vi "Smart IO Set Led Device Buffer.vi"(6 "force":bool, 8 "error in (no error)":errorcluster, 9 "buffer Data":u32[](array[colorbox]), 11 "deviceIndex":i32=-1) -> (0 "error out":errorcluster)   [LabVIEW 2023, in "MrcLib.lvlib"]
doc: "Update the LED color buffer for the wired device channel or leave device unwired if you choose to update the entire buffer in a single call."
uses:
  <vilib>/MRC/MrcLib.lvlib
  <vilib>/MRC/Types/MRC Smart IO Mode.ctl
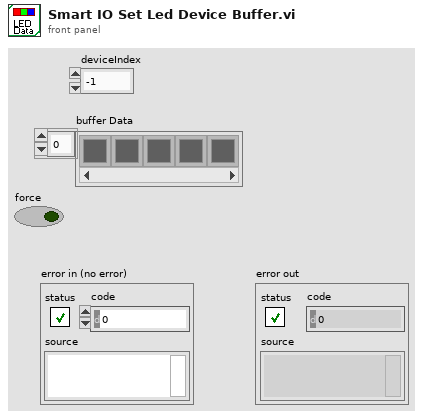
[diagram p1: front panel]
types:
  T1 = typedef "MRC Smart IO Mode.ctl" = i32
  T2 = enum16{"update device span", "update LED buffer", "clear"}
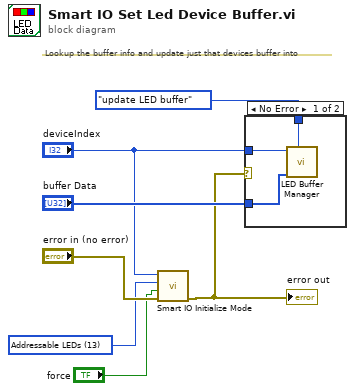
[diagram p0: block diagram]
diagram:
  w3 = T1 13 items=["Digital Input"=0, "Digital Output"=1, "Analog Input"=2, "PWM Input"=3, "PWM Output"=4, "Counter Rising"=5, "Counter Falling"=6, "Addressable LEDs"=13] ("mode")
  # "Lookup the buffer info and update just that devices buffer into"
  n1 = call <vilib>:"Smart IO Initialize Mode.vi"("error in (no error)"="error in (no error)", "force"="force", "mode"=w3, "deviceIndex"="deviceIndex") -> ("error out"=w1:errorcluster)  [unwired: 7 in]
  "error out" <- w1
  n2 = case shown="No Error" w1 {
    tunnel: "buffer Data" -> [w10 _]
    tunnel: T2."update LED buffer" ("action") -> [w9 _]
    tunnel: "deviceIndex" -> [w8 _]
    frame No Error {
      n3 = call <vilib>:"LED Buffer Manager.vi"("action"=w9, "Colors"=w10, "deviceIndex"=w8) -> ()  [unwired: 9 in]
    }
    frame Error {
    }
  }
